vi "Burst.vi"(0 "RFFE RegReadExt Command in":refnum<class "RFFE RegReadExt Command.lvclass">, 1 "Bus Number":i32, 5 "instrument handle in":refnum<k15>, 11 "error in (no error)":errorcluster) -> (4 "RFFE RegReadExt Command out":refnum<class "RFFE RegReadExt Command.lvclass">, 6 "instrument handle out":refnum<k15>, 15 "error out":errorcluster)   [LabVIEW 2018, in "MIPI RFFE API.lvlib" / "RFFE RegReadExt Command.lvclass"]
uses:
  RFFE RegReadExt Command.lvclass
  C:/Users/semoore/Projects/mipi-rffe-labview-oop/Extended Command/RFFE Extended Command.lvclass
  Extended Command/RFFE Extended Command.lvclass/RFFE Extended Command.ctl
  RFFE RegReadExt Command.lvclass/RFFE RegReadExt Command.ctl
  Extended Command/Set Register Data.vi
  Extended Command/RFFE Extended Command.lvclass
  MIPI RFFE API.lvlib
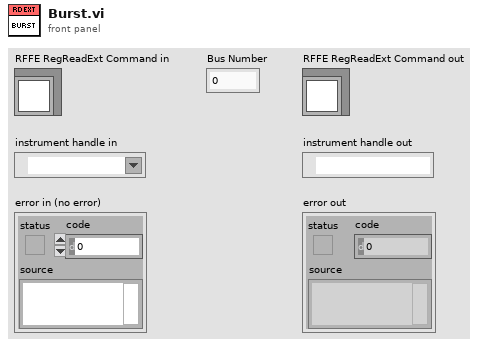
[diagram p1: front panel]
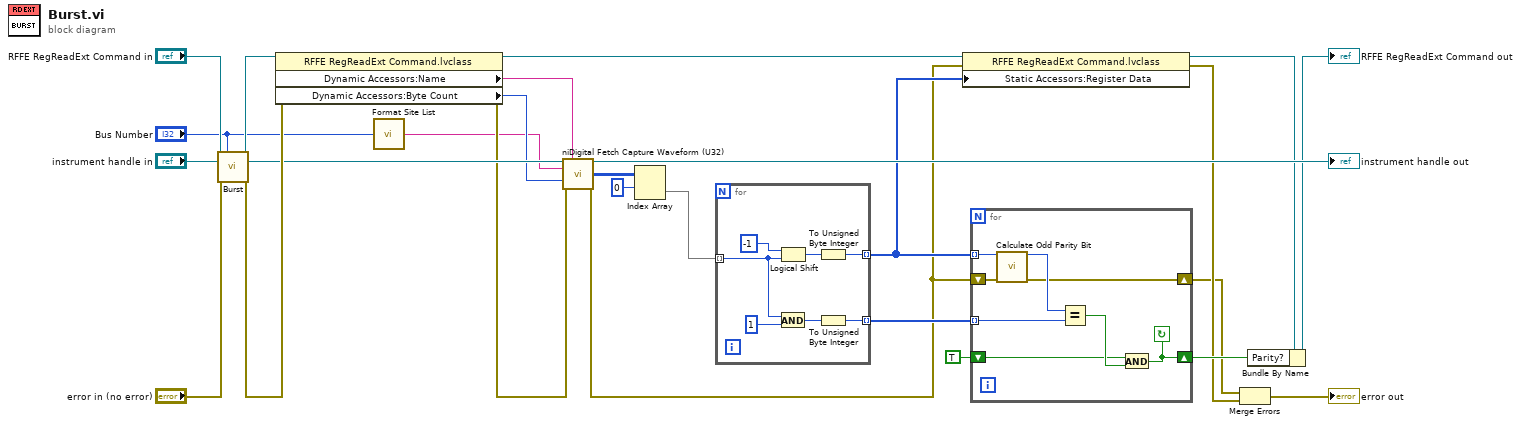
[diagram p0: block diagram]
diagram:
  n1 = call-parent "Burst.vi"("RFFE Command in"="RFFE RegReadExt Command in", "Bus Number"="Bus Number", "instrument handle in"="instrument handle in", "error in (no error)"="error in (no error)") -> ("RFFE Command out"=w25:refnum<class "RFFE RegReadExt Command.lvclass">, "instrument handle out"=w20:refnum<k15>, "error out"=w22:errorcluster)  [unwired: 9 in]
  n2 = property class="RFFE RegReadExt Command.lvclass"(reference=w25, error in=w22) -> (reference out=w16:refnum<class "RFFE RegReadExt Command.lvclass">, error out=w17:errorcluster, "Dynamic Accessors:Name"=w18:string, "Dynamic Accessors:Byte Count"=w13:i32)
  n3 = call "Format Site List.vi"("Bus Number"="Bus Number") -> ("Site List"=w12:string)  [unwired: 14 in]
  n4 = call <instrlib>:"niDigital Fetch Capture Waveform (U32).vi"("instrument handle"=w20, "waveform name"=w18, "site list"=w12, "samples to read"=w13, "error in"=w17) -> ("instrument handle out"=→"instrument handle out":refnum<k15>, "data"=w15:u32[][], "error out"=w8:errorcluster)  [unwired: 8 in]
  n5 = Index Array(array=w15, index (row)=0) -> (element=w11:u32[])  [unwired: 1 in]
  n6 = for {
    tunnel: w11 -> [w30] mode=indexing
    tunnel: [w28] -> w10 mode=indexing
    tunnel: [w27] -> w9 mode=indexing
    n7 = Logical Shift(y=i16 -1, x=w30) -> (x << y=w31:u32)
    n8 = And(x=w30, y=u32 1) -> (x .and. y?=w29:u32)
    n9 = To Unsigned Byte Integer(number=w31) -> (unsigned 8bit integer=w28:u8)
    n10 = To Unsigned Byte Integer(number=w29) -> (unsigned 8bit integer=w27:u8)
  }
  n11 = property class="RFFE RegReadExt Command.lvclass"(reference=w16, error in=w8, "Static Accessors:Register Data"=w10) -> (reference out=w6:refnum<class "RFFE RegReadExt Command.lvclass">, error out=w2:errorcluster)
  n12 = for {
    tunnel: w10 -> [w41] mode=indexing
    tunnel: w9 -> [w39] mode=indexing
    shift-right: [w38] -> w1
    shift-left: w8 -> [w37]
    shift-right: [w34] -> w4
    shift-left: TRUE -> [w35]
    stop <- w34 continue-if-true
    n13 = call "Calculate Odd Parity Bit.vi"("Byte"=w41, "error in (no error)"=w37) -> ("Odd Parity Bit"=w40:u8, "error out"=w38:errorcluster)  [unwired: 12 in]
    n14 = Equal?(x=w40, y=w39) -> (x = y?=w36:bool)
    n15 = And(x=w35, y=w36) -> (x .and. y?=w34:bool)
  }
  n16 = Merge Errors(w1, w2) -> (→"error out":errorcluster)
  n17 = Bundle By Name(cluster=w6, "Parity?"=w4) -> (→"RFFE RegReadExt Command out":refnum<class "RFFE RegReadExt Command.lvclass">)
